vi "OverlayRectangleCenterSize.vi"(4 "Color":u32(colorbox)=16711680, 5 "Angle":dbl, 6 "Drawing Mode (Frame)":T2, 7 "GroupName":string, 8 "error in":errorcluster, 9 "Size":T1, 10 "Center-Point":T1, 11 "Image Reference In":T3) -> (0 "error out":errorcluster, 3 "Image Reference Out":T3)   [LabVIEW 2020, in "OpenLvVision_Overlays.lvlib"]
doc: "Overlays an rectangle on top of an image.\nDraws the rectangle arround a center point."
uses:
  OpenLvVision_Overlays.lvlib
  <vilib>/OpenLvVision/OpenLvVision_Image/Management/TypeDef/OLV Image.ctl
  TypeDefs/DrawingMode.ctl
  TypeDefs/PointI32.ctl
  <vilib>/OpenLvVision/OpenLvVision_Image/Management/OLV Management.lvlib
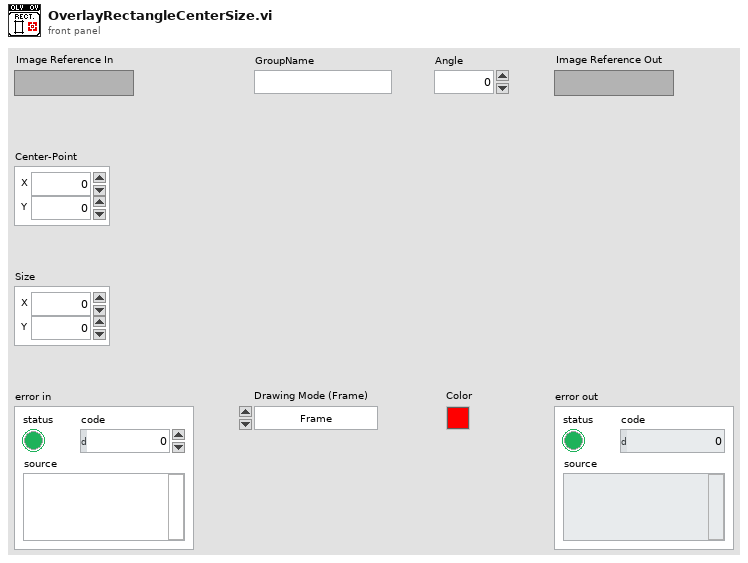
[diagram p1: front panel]
types:
  T1 = typedef "OpenLvVision_Overlays.lvlib/PointI32.ctl" = cluster{"X":i32, "Y":i32}
  T2 = typedef "OpenLvVision_Overlays.lvlib/DrawingMode.ctl" = enum16{"Frame", "Fill"}
  T3 = typedef "OLV OpenLvVision_Image.lvlib/OLV Management.lvlib/OLV Image.ctl" = refnum<image>
  T4 = typedef "OLV OpenLvVision_Image.lvlib/OLV DataAccess.lvlib/OLV RectangleI32.ctl" = cluster{"Left":i32, "Top":i32, "Right":i32, "Bottom":i32}
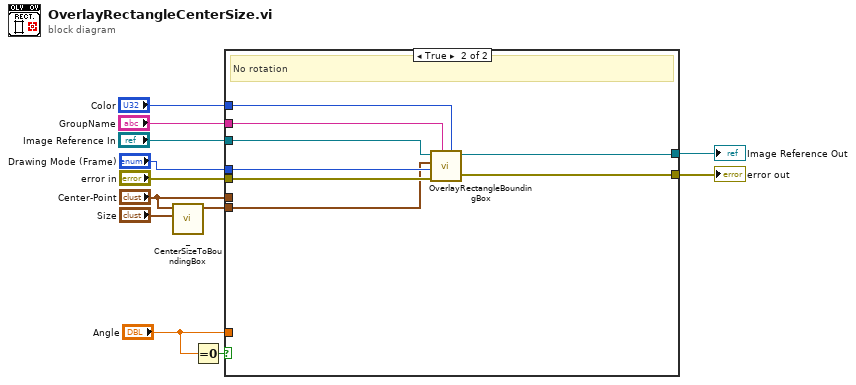
[diagram p0: block diagram]
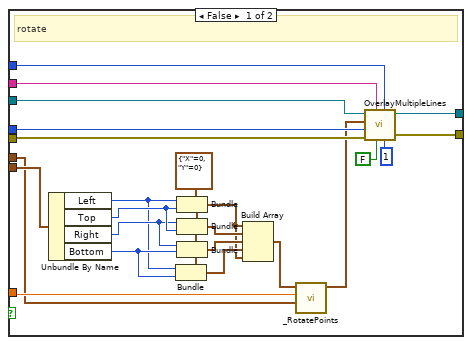
[diagram p2: hidden frame]
diagram:
  n1 = call "_CenterSizeToBoundingBox.vi"("Size"="Size", "Center-Point"="Center-Point") -> ("Bounding Box"=w2:T4)  [unwired: 9 in]
  n2 = Equal To 0?(x="Angle") -> (x = 0?=w3:bool)
  n3 = case shown="True" w3 {
    tunnel: [w14 w43] -> w12
    tunnel: [w13 w42] -> w11
    tunnel: "GroupName" -> [w15 w41]
    tunnel: "error in" -> [w33 w40]
    tunnel: "Drawing Mode (Frame)" -> [w32 w39]
    tunnel: "Image Reference In" -> [w34 w38]
    tunnel: "Color" -> [w28 w36]
    tunnel: "Angle" -> [w29 _]
    tunnel: w2 -> [w27 w37]
    tunnel: "Center-Point" -> [w26 _]
    frame False {
      w25 = T1 {"X"=0, "Y"=0} ("Origin")
      # "rotate"
      n4 = Unbundle By Name(w27) -> ("Left"=w17:i32, "Top"=w20:i32, "Right"=w19:i32, "Bottom"=w18:i32)
      n5 = Bundle(cluster=w25, "X"=w17, "Y"=w20) -> (w16:T1)
      n6 = Bundle(cluster=w16, "X"=w17, "Y"=w18) -> (w22:T1)
      n7 = Bundle(cluster=w25, "X"=w19, "Y"=w20) -> (w24:T1)
      n8 = Bundle(cluster=w16, "X"=w19, "Y"=w18) -> (w23:T1)
      n9 = Build Array(w16, w24, w23, w22, w16) -> (w21:T1[])
      n10 = call "_RotatePoints.vi"("Origin"=w26, "Angle"=w29, "Points in"=w21) -> ("Points out"=w30:T1[])  [unwired: 8 in]
      n11 = call "OverlayMultipleLines.vi"("Width"=u32 1, "Color"=w28, "Maintain Width?"=FALSE, "GroupName"=w15, "error in"=w33, "Drawing Mode (Frame)"=w32, "Points"=w30, "Image Reference In"=w34) -> ("error out"=w13:errorcluster, "Image Reference Out"=w14:T3)  [unwired: 2 in]
    }
    frame True {
      # "No rotation"
      n12 = call "OverlayRectangleBoundingBox.vi"("Color"=w36, "GroupName"=w41, "error in"=w40, "Drawing Mode (Frame)"=w39, "Rectangle"=w37, "Image Reference In"=w38) -> ("error out"=w42:errorcluster, "Image Reference Out"=w43:T3)  [unwired: 4 in]
    }
  }
  "error out" <- w11
  "Image Reference Out" <- w12
